vi "Carrier.vi"(0 "obj in":refnum<class "Sensor.lvclass">) -> (1 "obj out":refnum<class "Sensor.lvclass">)   [LabVIEW 2026, in "Sensor.lvclass"]
doc: "Round15 P15: STATIC pass-through member of Sensor. Its class-typed terminals are retyped by lvai_add_class_method WITHOUT dynamic dispatch, so calling it with a Temp Sensor constant leaves the link alone and puts a SENSOR-typed wire on obj out - the type launderer that makes runtime dispatch observable."
uses:
  Sensor.lvclass
  Sensor.lvclass/Sensor.ctl
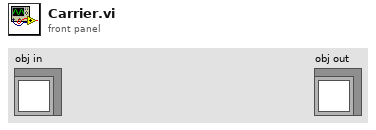
[diagram p1: front panel]
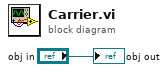
[diagram p0: block diagram]
diagram:
  "obj out" <- "obj in"
